vi "SQL_CHECK-Server.vi"(4 "Passwort":string, 6 "User Name":string, 8 "error in (no error)":errorcluster caption="Fehler (Eingang, kein Fehler)", 10 "Database Name":string, 11 "Server Name":string) -> (0 "error out":errorcluster caption="Fehler (Ausgang)", 1 "Server present?":bool, 2 "No User Right":bool, 3 "Server Connection OK":bool, 5 "Fehler Connection":errorcluster)   [LabVIEW 2024, in "DB-Tool.lvlib"]
doc: "Prüft die Erreichbarkeit eines Microsoft SQL Servers und die Gültigkeit der angegebenen Anmeldedaten. Das VI erstellt anhand der übergebenen Server-, Datenbank- und Benutzerdaten einen Connection-String und versucht eine Datenbankverbindung aufzubauen.\n\nStandardmäßig wird der zuvor ermittelte bzw. installierte Microsoft OLE DB Driver for SQL Server (MSOLEDBSQL) verwendet. Ist eine neuere Version vorhanden, wird diese bevorzugt verwendet (z. B. MSOLEDBSQL18 oder MSOLEDBSQL19).\n\nDas VI liefert Informationen über:\n\nErreichbarkeit des SQL-Servers\nErfolgreichen Verbindungsaufbau\nFehlende Benutzerberechtigungen\nVerwendeten Connection-String\nVerbindungsfehler\n\nVerwendungszweck:\n Vorprüfung für Datenbankverbindungen, um sicherzustellen, dass SQL-Server, Datenbank und Benutzerzugriff korrekt konfiguriert sind, bevor weitere Datenbankoperationen durchgeführt werden."
uses:
  DB-Tool.lvlib
  <vilib>/addons/database/Connection.llb/DB Tools Open Connec (String).vi
  <vilib>/addons/database/NI_Database_API.lvlib
panel:
  # "Connector Pane"
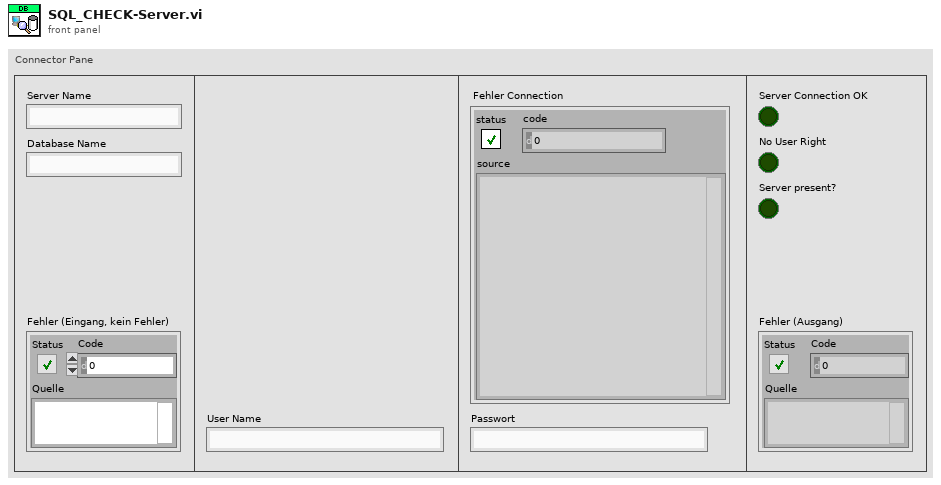
[diagram p1: front panel]
types:
  T1 = typedef "NI_Database_API.lvlib/Conn ObjectReference.ctl" = refnum<k1>
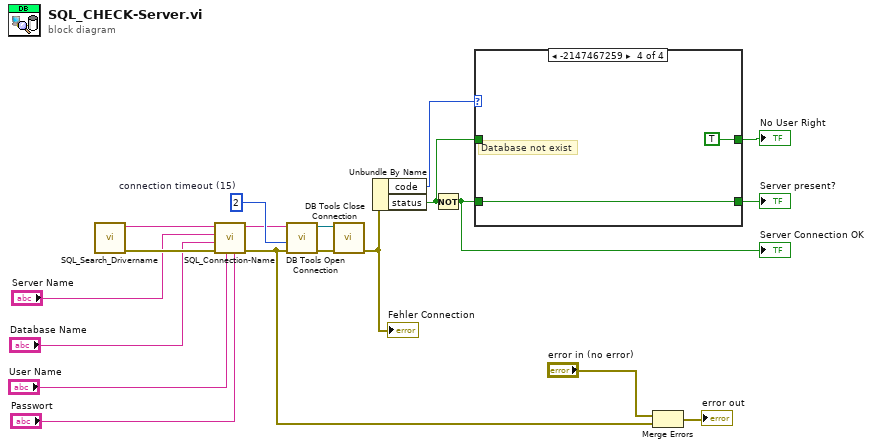
[diagram p0: block diagram]
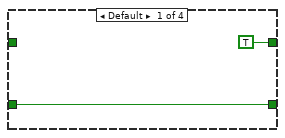
[diagram p2: hidden frame]
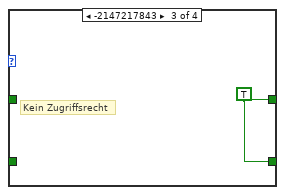
[diagram p4: hidden frame]
diagram:
  w17 = 2  # connection timeout (15)
  n1 = call "SQL_Search_Drivername.vi"() -> ("error out"=w9:errorcluster, "Client Name"=w10:string)  [unwired: 8 in, 2 out]
  n2 = call "SQL_Connection-Name.vi"("Passwort"="Passwort", "User Name"="User Name", "error in (no error)"=w9, "Database Name"="Database Name", "Server Name"="Server Name", "SQL Driver  Clientname"=w10) -> ("error out"=w8:errorcluster, "Connection String"=w4:string)  [unwired: 4 in]
  n3 = call-poly <vilib>:"DB Tools Open Connection.vi"("error in (no error)"=w8, "connection timeout (15)"=w17, "connection information"=w4) -> ("error out"=w19:errorcluster, "connection reference"=w18:T1)  [unwired: 5 in]
  n4 = call <vilib>:"DB Tools Close Connection.vi"("error in (no error)"=w19, "connection reference"=w18) -> ("error out"=w15:errorcluster)  [unwired: 5 in]
  "Fehler Connection" <- w15
  n5 = Unbundle By Name(w15) -> ("code"=w16:i32, "status"=w12:bool)
  n6 = Not(x=w12) -> (.not. x?=w5:bool)
  "Server Connection OK" <- w5
  n7 = case shown="-2147467259" w16 {
    tunnel: [TRUE w22 w24 TRUE] -> w14
    tunnel: w5 -> [w21 w23 _ w25]
    tunnel: [w21 w23 w24 w25] -> w13
    tunnel: w12 -> [_ w22 _ _]
    frame Default {
    }
    frame 0 {
    }
    frame -2147217843 {
      w24 = TRUE
      # "Kein Zugriffsrecht"
    }
    frame -2147467259 {
      # "Database not exist"
    }
  }
  "Server present?" <- w13
  "No User Right" <- w14
  n8 = Merge Errors("error in (no error)", w8) -> (→"error out":errorcluster)
